vi "Get Typedef Name.vi"(1 "embedded message name":string, 2 "generate serialization helpers":bool) -> (0 "typedef name":string)   [LabVIEW 2019, in "gRPC Template Creation Utility.lvlib"]
uses:
  gRPC Template Creation Utility.lvlib
  OneOf Constants/OneOfConstantsEnum.ctl
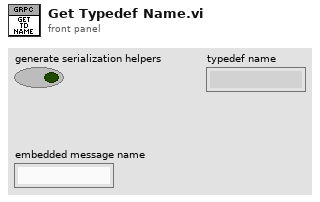
[diagram p1: front panel]
types:
  T1 = typedef "gRPC Template Creation Utility.lvlib/OneOfConstantsEnum.ctl" = enum16{"FlatToRichVIPrefix", "RichToFlatVIPrefix", "FlatTypeDefSuffix"}
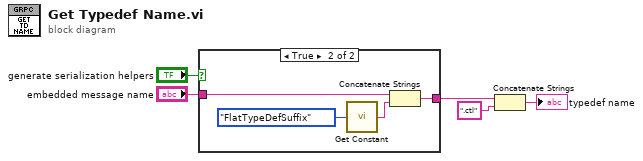
[diagram p0: block diagram]
diagram:
  n1 = case shown="True" "generate serialization helpers" {
    tunnel: "embedded message name" -> [w6 w10]
    tunnel: [w6 w9] -> w3
    frame False {
    }
    frame True {
      n2 = call "Get Constant.vi"("Selection"=OneOfConstantsEnum."FlatTypeDefSuffix") -> ("String"=w7:string)
      n3 = Concatenate Strings(w10, w7) -> (w9:string)
    }
  }
  n4 = Concatenate Strings(w3, ".ctl" ("string")) -> (→"typedef name":string)
